vi "Own20261012_SetNamedBundlerElements.vi"() -> ()   [LabVIEW 2024]
panel:
  out "error out":errorcluster caption="错误输出"
  in  "element_names":string[](array[string])
  in  "bundler_id":u32
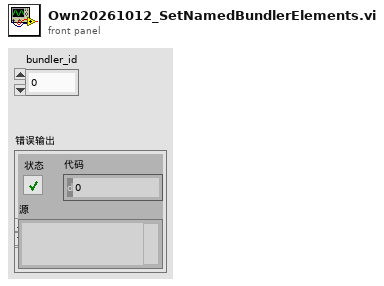
[diagram p1: front panel]
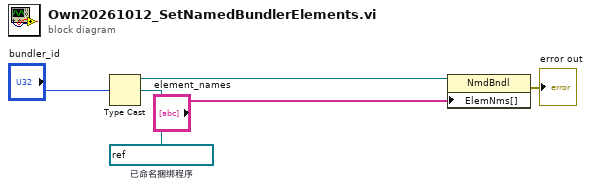
[diagram p0: block diagram]
diagram:
  w4 = refnum<vi> refnum  # 已命名捆绑程序
  n1 = Type Cast ("强制类型转换")(type=w4, x="bundler_id") -> (*(type *) &x=w3:refnum<vi>)
  n2 = property on="属性节点" class="NmdBndl"(reference=w3, "ElemNms[]"="element_names") -> (error out=→"error out":errorcluster)  [unwired: 1 in, 1 out]
